vi "Init.vi"(8 "error in":errorcluster, 10 "Sourcegrid Container":refnum<k24>(container), 11 "MyEventGrid in":refnum<class "MyEventGrid.lvclass">) -> (0 "error out":errorcluster, 3 "MyEventGrid out":refnum<class "MyEventGrid.lvclass">)   [LabVIEW 2026, in "MyEventGrid.lvclass"]
uses:
  MyEventGrid.lvclass
  source/Cells/Cell/Cell.lvclass
  source/Controllers/Custom Events/Custom Events.lvclass
  source/Editors/Combo Box/Combo Box.lvclass
  MyEventGrid.lvclass/MyEventGrid.ctl
  source/Grid/Set Column Default Width.vi
  source/Cells/Cell/Add Controller.vi
  source/Grid/SourceGrid.lvclass
  D:/git/Sourcegrid-LabVIEW/source/SourceGrid.dll
  source/SourceGrid.dll
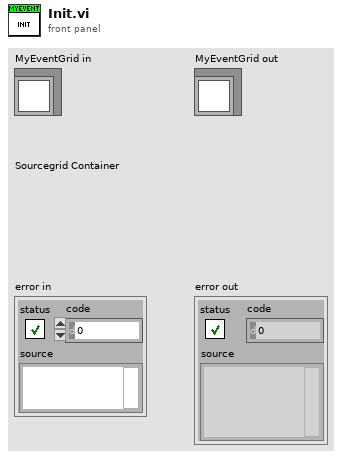
[diagram p1: front panel]
types:
  T1 = cluster{"onClick":refnum<user-event>, "onDoubleClick":refnum<user-event>, "onValueChanged":refnum<user-event>}
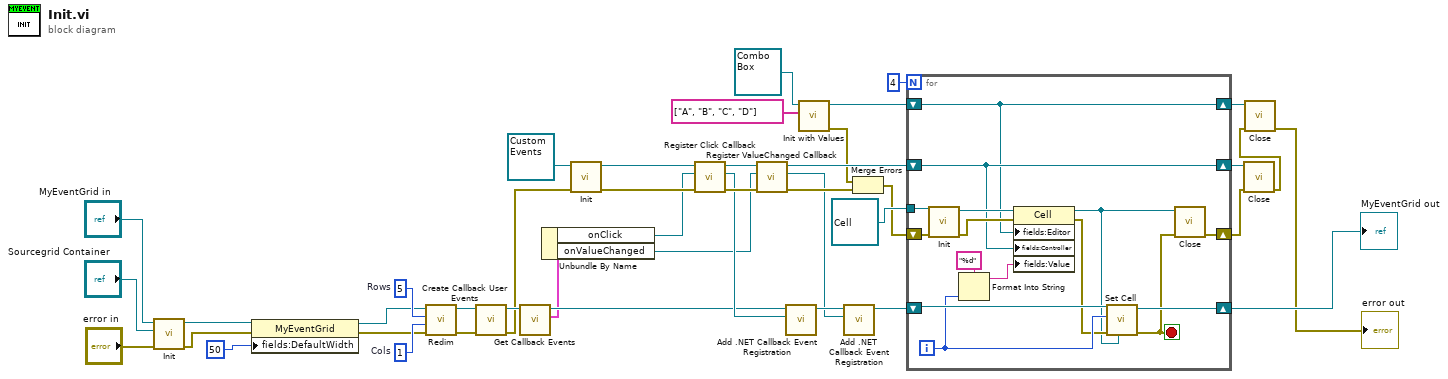
[diagram p0: block diagram]
diagram:
  w39 = 1  # Cols
  w40 = 5  # Rows
  n1 = call-parent "Init.vi"("error in"="error in", "Sourcegrid Container"="Sourcegrid Container", "Grid in"="MyEventGrid in") -> ("error out"=w31:errorcluster, "Grid out"=w30:refnum<class "MyEventGrid.lvclass">)  [unwired: 7 in]
  n2 = property class="MyEventGrid"(reference=w30, error in=w31, "fields:DefaultWidth"=50 ("DefaultWidth")) -> (reference out=w32:refnum<class "MyEventGrid.lvclass">, error out=w38:errorcluster)
  n3 = call "Redim.vi"("error in"=w38, "Columns"=w39, "Rows"=w40, "Sourcegrid in"=w32) -> ("error out"=w34:errorcluster, "Sourcegrid out"=w20:refnum<class "MyEventGrid.lvclass">)  [unwired: 6 in]
  n4 = call-dynamic "Create Callback User Events.vi"("error in"=w34, "MyEventGrid in"=w20) -> ("error out"=w15:errorcluster, "MyEventGrid out"=w19:refnum<class "MyEventGrid.lvclass">)  [unwired: 8 in]
  n5 = call "Get Callback Events.vi"("MyEventGrid in"=w19) -> ("Callback Events"=w17:T1, "MyEventGrid out"=w18:refnum<class "MyEventGrid.lvclass">)  [unwired: 9 in]
  n6 = Unbundle By Name(w17) -> ("onClick"=w16:refnum<user-event>, "onValueChanged"=w11:refnum<user-event>)
  n7 = call-dynamic "Init.vi"("error in"=w15, "Custom Events in"=refnum<class "Custom Events.lvclass"> refnum ("SourceGrid.lvlib:Custom Events.lvclass")) -> ("error out"=w25:errorcluster, "Custom Events out"=w23:refnum<class "Custom Events.lvclass">)  [unwired: 8 in]
  n8 = call-dynamic "Register Click Callback.vi"("error in"=w25, "onClick"=w16, "Custom Events in"=w23) -> ("error out"=w24:errorcluster, "Event Callback Refnum"=w22:refnum<k27>, "Custom Events out"=w13:refnum<class "Custom Events.lvclass">)  [unwired: 6 in]
  n9 = call-dynamic "Register ValueChanged Callback.vi"("error in"=w24, "onValueChanged"=w11, "Custom Events in"=w13) -> ("error out"=w14:errorcluster, "Event Callback Refnum"=w9:refnum<k27>, "Custom Events out"=w12:refnum<class "Custom Events.lvclass">)  [unwired: 6 in]
  n10 = call "Add .NET Callback Event Registration.vi"("Event Callback Refnum"=w22, "SourceGrid in"=w18) -> ("SourceGrid out"=w21:refnum<class "MyEventGrid.lvclass">)  [unwired: 9 in]
  n11 = call-dynamic "Init with Values.vi"("Values"=string[] ["A", "B", "C", "D"], "Combo Box in"=refnum<class "Combo Box.lvclass"> refnum ("SourceGrid.lvlib:Combo Box.lvclass")) -> ("error out"=w4:errorcluster, "Combo Box out"=w6:refnum<class "Combo Box.lvclass">)  [unwired: 8 in]
  n12 = call "Add .NET Callback Event Registration.vi"("Event Callback Refnum"=w9, "SourceGrid in"=w21) -> ("SourceGrid out"=w10:refnum<class "MyEventGrid.lvclass">)  [unwired: 9 in]
  n13 = Merge Errors(w4, w14) -> (w5:errorcluster)
  n14 = for {
    N: 4 -> [_]
    shift-right: [w47] -> w26
    shift-left: w5 -> [w48]
    shift-right: [w57] -> w28
    shift-left: w10 -> [w56]
    tunnel: refnum<class "Cell.lvclass"> refnum ("Cell in") -> [w52]
    shift-right: [w45] -> w27
    shift-left: w12 -> [w45]
    shift-right: [w44] -> w3
    shift-left: w6 -> [w44]
    i -> [w54]
    stop <- w49 stop-if-true
    n15 = call-dynamic "Init.vi"("error in"=w48, "Cell in"=w52) -> ("error out"=w50:errorcluster, "Cell out"=w51:refnum<class "Cell.lvclass">)  [unwired: 8 in]
    n16 = Format Into String(format string="%d", w54) -> (resulting string=w46:string)  [unwired: 2 in, 1 out]
    n17 = property class="Cell"(reference=w51, error in=w50, "fields:Editor"=w44, "fields:Controller"=w45, "fields:Value"=w46) -> (reference out=w43:refnum<class "Cell.lvclass">, error out=w53:errorcluster)
    n18 = call "Set Cell.vi"("Cell"=w43, "error in"=w53, "Row"=w54, "Sourcegrid in"=w56) -> ("error out"=w49:errorcluster, "Sourcegrid out"=w57:refnum<class "MyEventGrid.lvclass">)  [unwired: 6 in]
    n19 = call-dynamic "Close.vi"("error in"=w49, "Cell in"=w43) -> ("error out"=w47:errorcluster)  [unwired: 8 in, 1 out]
  }
  "MyEventGrid out" <- w28
  n20 = call-dynamic "Close.vi"("error in"=w26, "Custom Events in"=w27) -> ("error out"=w2:errorcluster)  [unwired: 8 in, 1 out]
  n21 = call-dynamic "Close.vi"("error in"=w2, "Combo Box in"=w3) -> ("error out"=→"error out":errorcluster)  [unwired: 8 in, 1 out]
